vi "ASD STD for Threshold VI.vi"(8 "S Point":i32=10, 11 "STD A":dbl[](array[numeric])) -> (3 "STD for Thd":dbl)   [LabVIEW 2018]
panel:
  out "サイズ":i32
  out "Y out":dbl[](array[numeric])
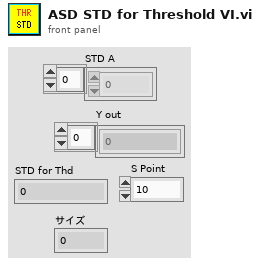
[diagram p1: front panel]
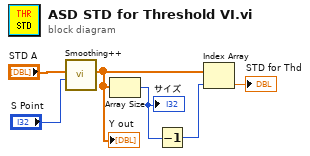
[diagram p0: block diagram]
diagram:
  n1 = call "Smoothing++.vi"("+/- Point"="S Point", "Y in"="STD A") -> ("Y out"=w4:dbl[])  [unwired: 9 in]
  "Y out" <- w4
  n2 = Array Size(array=w4) -> (size(s)=w3:i32)
  "サイズ" <- w3
  n3 = Decrement(x=w3) -> (x-1=w1:i32)
  n4 = Index Array(array=w4, index=w1) -> (element=→"STD for Thd":dbl)
